vi "Write Batch Values - Double.vi"(8 "error in (no error)":errorcluster, 10 "Array":dbl[](array[numeric]), 11 "OD Batch in":refnum<class "OD Batch.lvclass">) -> (0 "error out":errorcluster, 3 "OD Batch out":refnum<class "OD Batch.lvclass">)   [LabVIEW 2023, in "xnet_canopen.lvlib" / "OD Batch.lvclass"]
doc: "Expect OD Vars are all numeric types.\n\nFor I64 and U64, use <b>Type Cast</b> to restore exact value from double; For other types, use directly conversion."
uses:
  OD Batch.lvclass
  OD Batch.lvclass/OD Batch.ctl
  Write Batch OD By Array Index - u8.vi
  Write Batch OD By Array Index - i64.vi
  Write Batch OD By Array Index - bool.vi
  Write Batch OD By Array Index - f32.vi
  Write Batch OD By Array Index - i16.vi
  Write Batch OD By Array Index - u16.vi
  Write Batch OD By Array Index - i8.vi
  Write Batch OD By Array Index - u32.vi
  Write Batch OD By Array Index - u64.vi
  Write Batch OD By Array Index - i32.vi
  Write Batch OD By Array Index - f64.vi
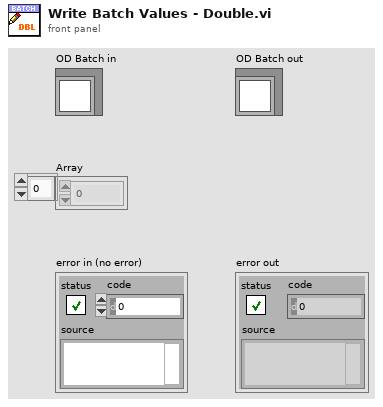
[diagram p1: front panel]
types:
  T1 = typedef "xnet_canopen.lvlib/od entry.ctl" = cluster{"OD Index":T2, "CANOpen Types":T3, "Size":u32, "Offset":u32, "Value":variant, "Initialized":bool}
  T2 = typedef "xnet_canopen.lvlib/od index.ctl" = cluster{"Index":u16, "SubIndex":u8}
  T3 = typedef "xnet_canopen.lvlib/canopen types.ctl" = u32
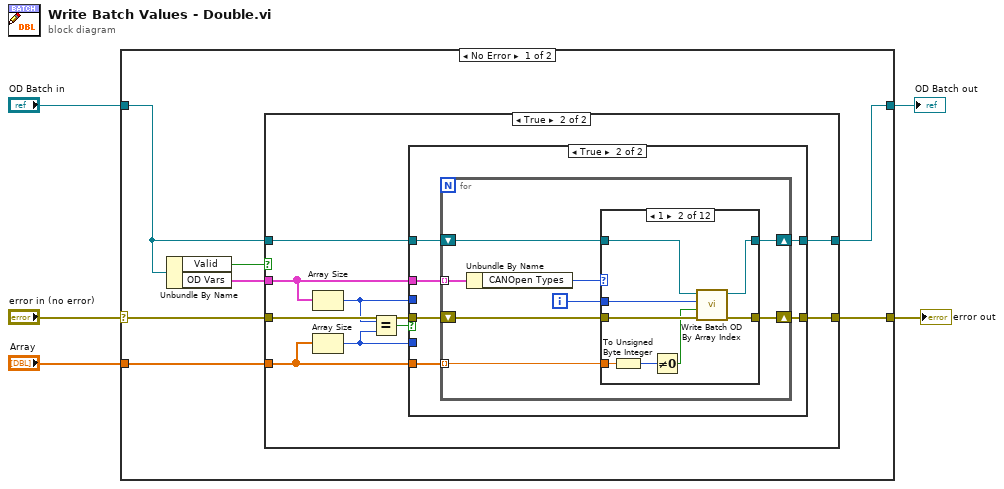
[diagram p0: block diagram]
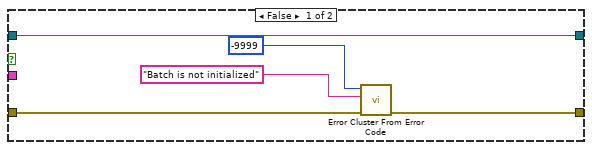
[diagram p2: hidden frame]
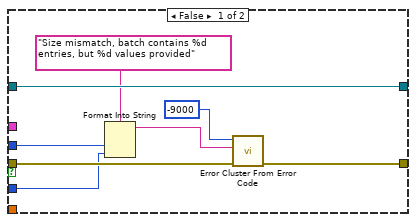
[diagram p3: hidden frame]
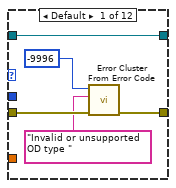
[diagram p4: hidden frame]
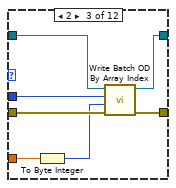
[diagram p5: hidden frame]
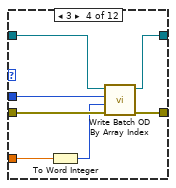
[diagram p6: hidden frame]
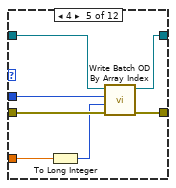
[diagram p7: hidden frame]
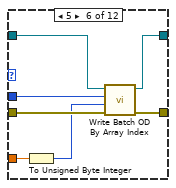
[diagram p8: hidden frame]
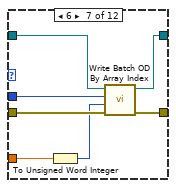
[diagram p9: hidden frame]
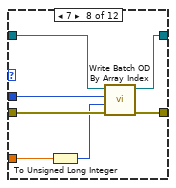
[diagram p10: hidden frame]
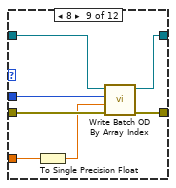
[diagram p11: hidden frame]
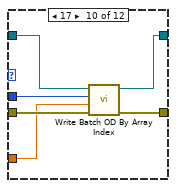
[diagram p12: hidden frame]
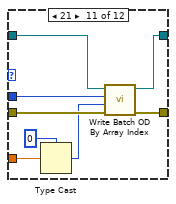
[diagram p13: hidden frame]
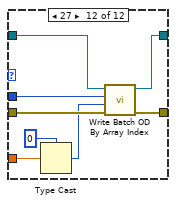
[diagram p14: hidden frame]
diagram:
  n1 = case shown="No Error" "error in (no error)" {
    selector: "error in (no error)" -> [w12 w133]
    tunnel: [w11 w133] -> w4
    tunnel: [w6 w134] -> w2
    tunnel: "OD Batch in" -> [w9 w134]
    tunnel: "Array" -> [w7 _]
    frame No Error {
      n2 = Unbundle By Name(w9) -> ("Valid"=w8:bool, "OD Vars"=w10:T1[])
      n3 = case shown="True" w8 {
        tunnel: w12 -> [w15 w26]
        tunnel: [w14 w25] -> w11
        tunnel: w10 -> [_ w22]
        tunnel: w9 -> [w13 w24]
        tunnel: w7 -> [_ w21]
        tunnel: [w13 w23] -> w6
        frame False {
          n4 = call <vilib>:"Error Cluster From Error Code.vi"("error in (no error)"=w15, "error message (\"\")"="Batch is not initialized" ("error message (\"\")"), "error code (0)"=-9999) -> ("error out"=w14:errorcluster)  [unwired: 6 in]
        }
        frame True {
          n5 = Array Size(array=w22) -> (size(s)=w18:i32)
          n6 = Array Size(array=w21) -> (size(s)=w19:i32)
          n7 = Equal?(x=w18, y=w19) -> (x = y?=w20:bool)
          n8 = case shown="True" w20 {
            tunnel: w26 -> [w34 w40]
            tunnel: [w32 w39] -> w25
            tunnel: w22 -> [_ w38]
            tunnel: w24 -> [w33 w37]
            tunnel: w21 -> [_ w36]
            tunnel: [w33 w35] -> w23
            tunnel: w19 -> [w29 _]
            tunnel: w18 -> [w28 _]
            frame False {
              n9 = Format Into String(format string="Size mismatch, batch contains %d entries, but %d values provided", w28, w29) -> (resulting string=w27:string)  [unwired: 2 in, 1 out]
              n10 = call <vilib>:"Error Cluster From Error Code.vi"("error in (no error)"=w34, "error message (\"\")"=w27, "error code (0)"=-9000) -> ("error out"=w32:errorcluster)  [unwired: 6 in]
            }
            frame True {
              n11 = for {
                shift-right: [w47] -> w39
                shift-left: w40 -> [w48]
                tunnel: w38 -> [w46] mode=indexing
                shift-right: [w41] -> w35
                shift-left: w37 -> [w43]
                tunnel: w36 -> [w42] mode=indexing
                i -> [w44]
                n12 = Unbundle By Name(w46) -> ("CANOpen Types"=w45:T3)
                n13 = case shown="1" w45 {
                  tunnel: w48 -> [w53 w61 w68 w75 w82 w89 w96 w103 w110 w116 w124 w132]
                  tunnel: [w52 w60 w67 w74 w81 w88 w95 w102 w109 w115 w123 w131] -> w47
                  tunnel: w44 -> [_ w59 w66 w73 w80 w87 w94 w101 w108 w114 w122 w130]
                  tunnel: w43 -> [w49 w58 w65 w72 w79 w86 w93 w100 w107 w113 w121 w129]
                  tunnel: w42 -> [_ w55 w64 w71 w78 w84 w92 w99 w106 w112 w117 w127]
                  tunnel: [w49 w54 w62 w69 w76 w85 w90 w97 w104 w111 w119 w125] -> w41
                  frame Default {
                    n14 = call <vilib>:"Error Cluster From Error Code.vi"("error in (no error)"=w53, "error message (\"\")"="Invalid or unsupported OD type " ("error message (\"\")"), "error code (0)"=-9996) -> ("error out"=w52:errorcluster)  [unwired: 6 in]
                  }
                  frame 1 {
                    n15 = To Unsigned Byte Integer(number=w55) -> (unsigned 8bit integer=w57:u8)
                    n16 = Not Equal To 0?(x=w57) -> (x != 0?=w56:bool)
                    n17 = call-poly "Write Batch OD By Array Index.vi"("error in (no error)"=w61, "value"=w56, "array index"=w59, "OD Batch in"=w58) -> ("error out"=w60:errorcluster, "OD Batch out"=w54:refnum<class "OD Batch.lvclass">)  [unwired: 6 in]
                  }
                  frame 2 {
                    n18 = To Byte Integer(number=w64) -> (8bit integer=w63:i8)
                    n19 = call-poly "Write Batch OD By Array Index.vi"("error in (no error)"=w68, "value"=w63, "array index"=w66, "OD Batch in"=w65) -> ("error out"=w67:errorcluster, "OD Batch out"=w62:refnum<class "OD Batch.lvclass">)  [unwired: 6 in]
                  }
                  frame 3 {
                    n20 = To Word Integer(number=w71) -> (16bit integer=w70:i16)
                    n21 = call-poly "Write Batch OD By Array Index.vi"("error in (no error)"=w75, "value"=w70, "array index"=w73, "OD Batch in"=w72) -> ("error out"=w74:errorcluster, "OD Batch out"=w69:refnum<class "OD Batch.lvclass">)  [unwired: 6 in]
                  }
                  frame 4 {
                    n22 = To Long Integer(number=w78) -> (32bit integer=w77:i32)
                    n23 = call-poly "Write Batch OD By Array Index.vi"("error in (no error)"=w82, "value"=w77, "array index"=w80, "OD Batch in"=w79) -> ("error out"=w81:errorcluster, "OD Batch out"=w76:refnum<class "OD Batch.lvclass">)  [unwired: 6 in]
                  }
                  frame 5 {
                    n24 = To Unsigned Byte Integer(number=w84) -> (unsigned 8bit integer=w83:u8)
                    n25 = call-poly "Write Batch OD By Array Index.vi"("error in (no error)"=w89, "value"=w83, "array index"=w87, "OD Batch in"=w86) -> ("error out"=w88:errorcluster, "OD Batch out"=w85:refnum<class "OD Batch.lvclass">)  [unwired: 6 in]
                  }
                  frame 6 {
                    n26 = To Unsigned Word Integer(number=w92) -> (unsigned 16bit integer=w91:u16)
                    n27 = call-poly "Write Batch OD By Array Index.vi"("error in (no error)"=w96, "value"=w91, "array index"=w94, "OD Batch in"=w93) -> ("error out"=w95:errorcluster, "OD Batch out"=w90:refnum<class "OD Batch.lvclass">)  [unwired: 6 in]
                  }
                  frame 7 {
                    n28 = To Unsigned Long Integer(number=w99) -> (unsigned 32bit integer=w98:u32)
                    n29 = call-poly "Write Batch OD By Array Index.vi"("error in (no error)"=w103, "value"=w98, "array index"=w101, "OD Batch in"=w100) -> ("error out"=w102:errorcluster, "OD Batch out"=w97:refnum<class "OD Batch.lvclass">)  [unwired: 6 in]
                  }
                  frame 8 {
                    n30 = To Single Precision Float(number=w106) -> (single precision float=w105:sgl)
                    n31 = call-poly "Write Batch OD By Array Index.vi"("error in (no error)"=w110, "value"=w105, "array index"=w108, "OD Batch in"=w107) -> ("error out"=w109:errorcluster, "OD Batch out"=w104:refnum<class "OD Batch.lvclass">)  [unwired: 6 in]
                  }
                  frame 17 {
                    n32 = call-poly "Write Batch OD By Array Index.vi"("error in (no error)"=w116, "value"=w112, "array index"=w114, "OD Batch in"=w113) -> ("error out"=w115:errorcluster, "OD Batch out"=w111:refnum<class "OD Batch.lvclass">)  [unwired: 6 in]
                  }
                  frame 21 {
                    n33 = Type Cast(type=i64 0, x=w117) -> (*(type *) &x=w118:i64)
                    n34 = call-poly "Write Batch OD By Array Index.vi"("error in (no error)"=w124, "value"=w118, "array index"=w122, "OD Batch in"=w121) -> ("error out"=w123:errorcluster, "OD Batch out"=w119:refnum<class "OD Batch.lvclass">)  [unwired: 6 in]
                  }
                  frame 27 {
                    n35 = Type Cast(type=u64 0, x=w127) -> (*(type *) &x=w126:u64)
                    n36 = call-poly "Write Batch OD By Array Index.vi"("error in (no error)"=w132, "value"=w126, "array index"=w130, "OD Batch in"=w129) -> ("error out"=w131:errorcluster, "OD Batch out"=w125:refnum<class "OD Batch.lvclass">)  [unwired: 6 in]
                  }
                }
              }
            }
          }
        }
      }
    }
    frame Error {
    }
  }
  "error out" <- w4
  "OD Batch out" <- w2
